vi "Selfcheck Negative Control.vi"() -> (0 "AllPass":bool, 1 "Total Error":dbl)   [LabVIEW 2026]
doc: "Round-13 self-contained test, no third-party framework: three static Calls to Conpane Probe B.vi, each result minus its expected value, the three residuals summed, and the sum compared with 0. Every case is exact in IEEE754 (3*5, -2*4, 0*7), so the sum is exactly 0 iff the subject is right. AllPass and Total Error are both on the connector pane, so a runner can read them like any other VI's outputs."
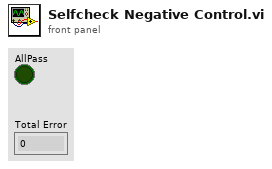
[diagram p1: front panel]
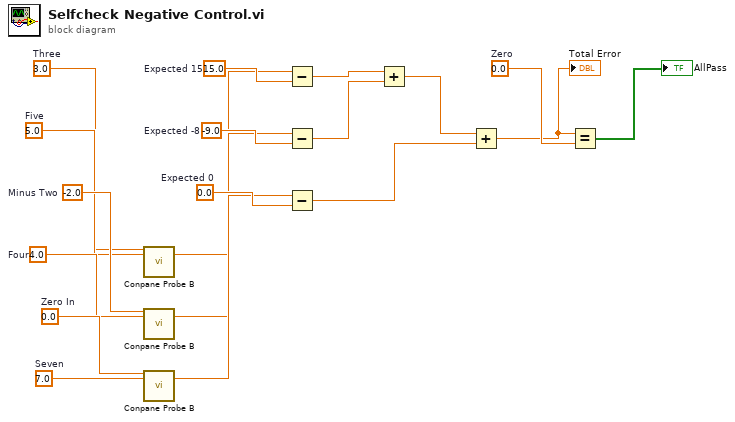
[diagram p0: block diagram]
diagram:
  w18 = 0.0  # Zero
  w14 = 0.0  # Expected 0
  w12 = 7.0  # Seven
  w11 = 0.0  # Zero In
  w9 = -9.0  # Expected -8
  w7 = 4.0  # Four
  w6 = -2.0  # Minus Two
  w4 = 15.0  # Expected 15
  w2 = 5.0  # Five
  w1 = 3.0  # Three
  n1 = call "Conpane Probe B.vi"("x"=w1, "factor"=w2) -> ("y"=w3:dbl)  [unwired: 13 in]
  n2 = call "Conpane Probe B.vi"("x"=w6, "factor"=w7) -> ("y"=w8:dbl)  [unwired: 13 in]
  n3 = call "Conpane Probe B.vi"("x"=w11, "factor"=w12) -> ("y"=w13:dbl)  [unwired: 13 in]
  n4 = Subtract(x=w3, y=w4) -> (x-y=w5:dbl)
  n5 = Subtract(x=w8, y=w9) -> (x-y=w10:dbl)
  n6 = Subtract(x=w13, y=w14) -> (x-y=w15:dbl)
  n7 = Add(x=w5, y=w10) -> (x+y=w16:dbl)
  n8 = Add(x=w16, y=w15) -> (x+y=w17:dbl)
  "Total Error" <- w17
  n9 = Equal?(x=w17, y=w18) -> (x = y?=→"AllPass":bool[])
